vi "Shutdown Sine Generator.vi"(8 "error in":errorcluster, 11 "next start sample":dbl) -> (0 "error out":errorcluster, 3 "samples elapsed":dbl)   [LabVIEW 2026, in "Sine Generator.lvlib"]
doc: "Shutdown stage. Finalises a generation run when the client cancels or an error stops the acquisition loop and reports the number of samples elapsed. The simulator holds no hardware sessions, files or other resources, so nothing needs to be closed; this is the single place to release resources if the engine ever acquires any."
uses:
  Sine Generator.lvlib
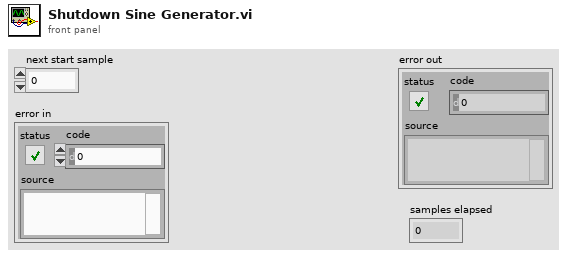
[diagram p1: front panel]
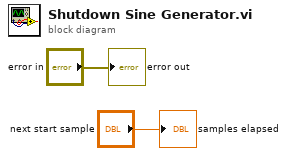
[diagram p0: block diagram]
diagram:
  "error out" <- "error in"
  "samples elapsed" <- "next start sample"
